vi "Reinit CAN Channel.vi"(8 "error in (no error)":errorcluster, 10 "Configuration.Frames to read":i32, 11 "CAN_Reader_NIXNET":refnum<class "CAN_Reader_CANsub_Plugin.lvclass">) -> (0 "error out":errorcluster, 3 "CAN_Reader_NIXNET":refnum<class "CAN_Reader_CANsub_Plugin.lvclass">)   [LabVIEW 2021, in "CAN_Reader_CANsub_Plugin.lvclass"]
uses:
  CAN_Reader_CANsub_Plugin.lvclass
  CAN_Reader_CANsub_Plugin.lvclass/CAN_Reader_CANsub_Plugin.ctl
  <vilib>/CIF Foundation/CIF Channels Core/ChannelCommon/typedef/FIFO Flags.ctl
  <vilib>/CIF Foundation/CIF Channels Core/ChannelCommon/ChannelCommon.lvlib
  <vilib>/CIF Foundation/CIF Core/CIFCore/Class/CIFCorePlugin.lvclass
  Common/Typedef/Channels.ctl
  Common/CAN_Reader_CANsub_Common.lvlib
  <vilib>/CIF Foundation/CIF Channels Core/ChannelCommon/typedef/New FIFO Config.ctl
  C:/Program Files/National Instruments/LabVIEW 2021/vi.lib/CIF Foundation/CIF Core/CIFCore/Class/CIFCorePlugin.lvclass
  D:/dev/Plugins/CAN_Reader_CANsub/Class/CAN_Reader_CANsub_Plugin.lvclass
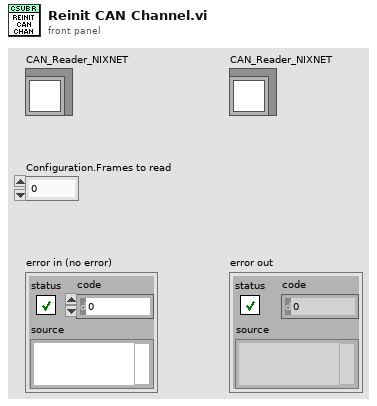
[diagram p1: front panel]
types:
  T1 = typedef "ChannelCommon.lvlib/New FIFO Config.ctl" = cluster{"Max Bytes/Msg":u64, "Max Msg/FIFO":u64, "FIFO Flags":T2}
  T2 = typedef "ChannelCommon.lvlib/FIFO Flags.ctl" = cluster{"Backpressure":bool}
  T3 = typedef "CAN_Reader_CANsub_Common.lvlib/Channels.ctl" = enum16{"CAN_Frames"}
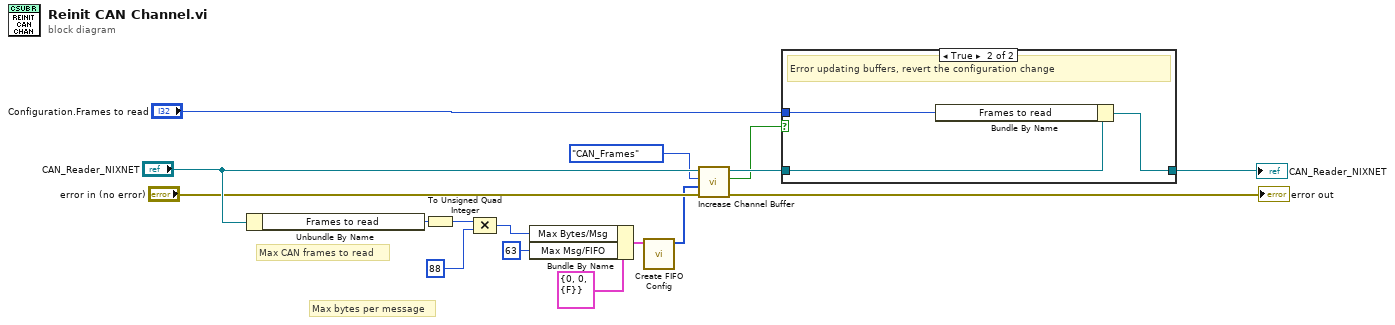
[diagram p0: block diagram]
diagram:
  # "Max bytes per message"
  # "Max CAN frames to read"
  n1 = Unbundle By Name("CAN_Reader_NIXNET") -> ("Frames to read"=w2:i32)
  n2 = To Unsigned Quad Integer(1:w2) -> (0:w3:u64)
  n3 = Compound Arithmetic op=MULTIPLY(w3, u64 88 ("Max Msg/FIFO")) -> (w1:u64)
  n4 = Bundle By Name(cluster=T1 {"Max Bytes/Msg"=0, "Max Msg/FIFO"=0, "FIFO Flags"={"Backpressure"=FALSE}} ("New FIFO Config"), "Max Bytes/Msg"=w1, "Max Msg/FIFO"=u64 63) -> (w8:T1)
  n5 = call <vilib>:"Create FIFO Config.vi"("New FIFO Config"=w8) -> ("Flattened FIFO Config"=w4:u8[])  [unwired: 10 in]
  n6 = call <vilib>:"Increase Channel Buffer.vi"("error in (no error)"="error in (no error)", "Flattened FIFO Config"=w4, "Channel Index"=Channels."CAN_Frames" ("Channels"), "CIFCorePlugin in"="CAN_Reader_NIXNET") -> ("error out"=→"error out":errorcluster, "Error Increasing Buffer"=w10:bool, "CIFCorePlugin out"=w15:refnum<class "CAN_Reader_CANsub_Plugin.lvclass">)  [unwired: 5 in]
  n7 = case shown="True" w10 {
    tunnel: w15 -> [w17 w20]
    tunnel: [w17 w19] -> w14
    tunnel: "Configuration.Frames to read" -> [_ w18]
    frame False {
      # "No error updating buffers"
    }
    frame True {
      # "Error updating buffers, revert the configuration change"
      n8 = Bundle By Name(cluster=w20, "Frames to read"=w18) -> (w19:refnum<class "CAN_Reader_CANsub_Plugin.lvclass">)
    }
  }
  "CAN_Reader_NIXNET" <- w14
